vi "Digital_Write.vi"(8 "error in (no error)":errorcluster, 9 "Valor":bool, 10 "Canal":u8, 11 "VISA resource name":refnum<visa-resource-name>) -> (0 "error out":errorcluster, 2 "respuesta":string, 3 "VISA resource name out":refnum<visa-resource-name>)   [LabVIEW 2026]
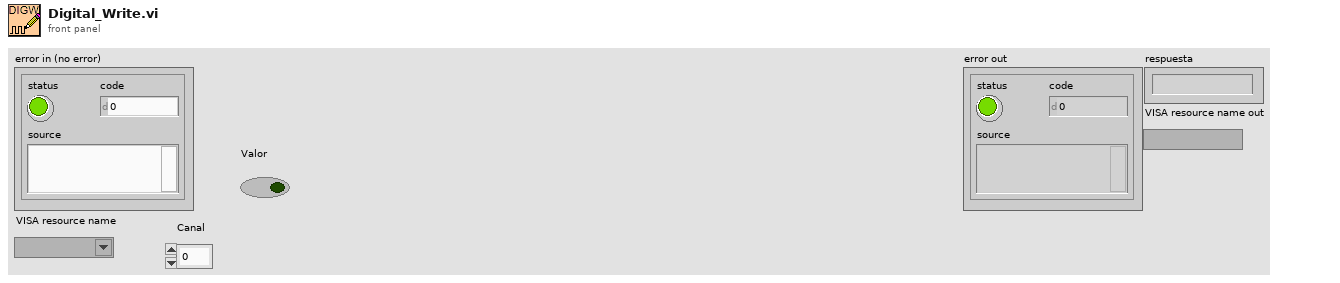
[diagram p1: front panel]
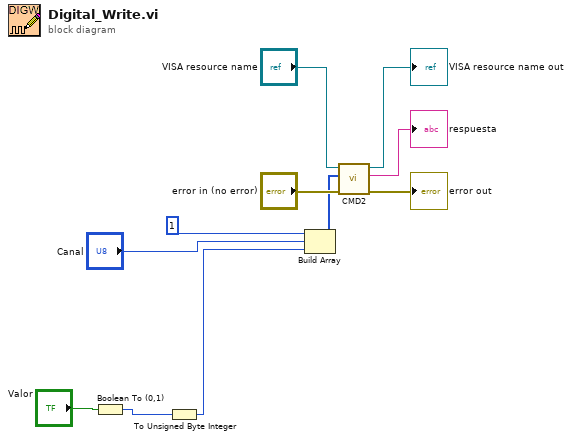
[diagram p0: block diagram]
diagram:
  n1 = Boolean To (0,1)(Boolean="Valor") -> (0, 1=w4:i16)
  n2 = To Unsigned Byte Integer(number=w4) -> (unsigned 8bit integer=w3:u8)
  n3 = Build Array(u8 1 ("Numeric"), "Canal", w3) -> (w1:u8[])
  n4 = call "CMD2.vi"("error in (no error)"="error in (no error)", "Comando"=w1, "VISA resource name"="VISA resource name") -> ("error out"=→"error out":errorcluster, "respuesta"=→"respuesta":string, "VISA resource name out"=→"VISA resource name out":refnum<visa-resource-name>)  [unwired: 6 in]
